vi "Localize CSM VIs.vi"(5 "API Dir":path[](array[path]), 6 "options":cluster{"Force?(F)":bool, "Show FP":bool}={"Force?(F)"=FALSE, "Show FP"=TRUE}, 7 "doc dir":path[](array[path]), 8 "error in (no error)":errorcluster, 10 "Language Ring":string(combo)="English(en-us)") -> (0 "error out":errorcluster)   [LabVIEW 2017, in "csmdoc.lvlib"]
uses:
  csmdoc.lvlib
  BEditor-Localization.vi
  _Typedef/DocElement.ctl
  _Shared/CSM Shared.lvlib
  _tool/_batchEditorDialog/batchEditorDialog.lvlib
  Communicable State Machine.lvlib
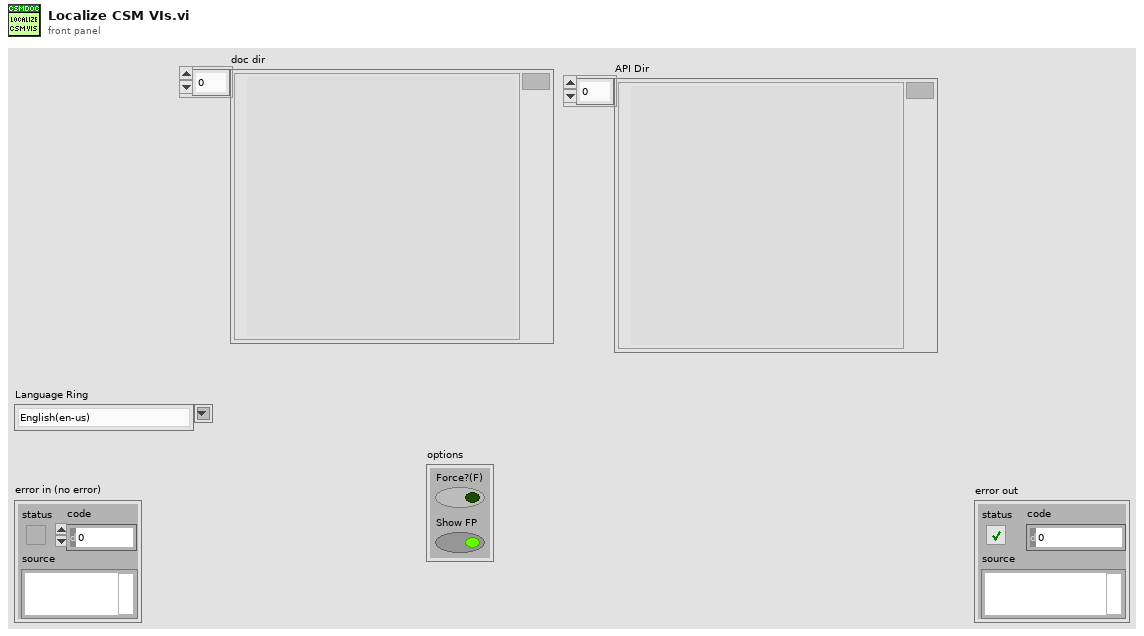
[diagram p1: front panel]
types:
  T1 = typedef "csmdoc.lvlib/DocNote.ctl" = cluster{"ID":string, "Content":string, "Type":string}
  T2 = typedef "csmdoc.lvlib/DocElement.ctl" = cluster{"ID":string, "Content":string[], "SubIDs":string[], "Path":string[]}
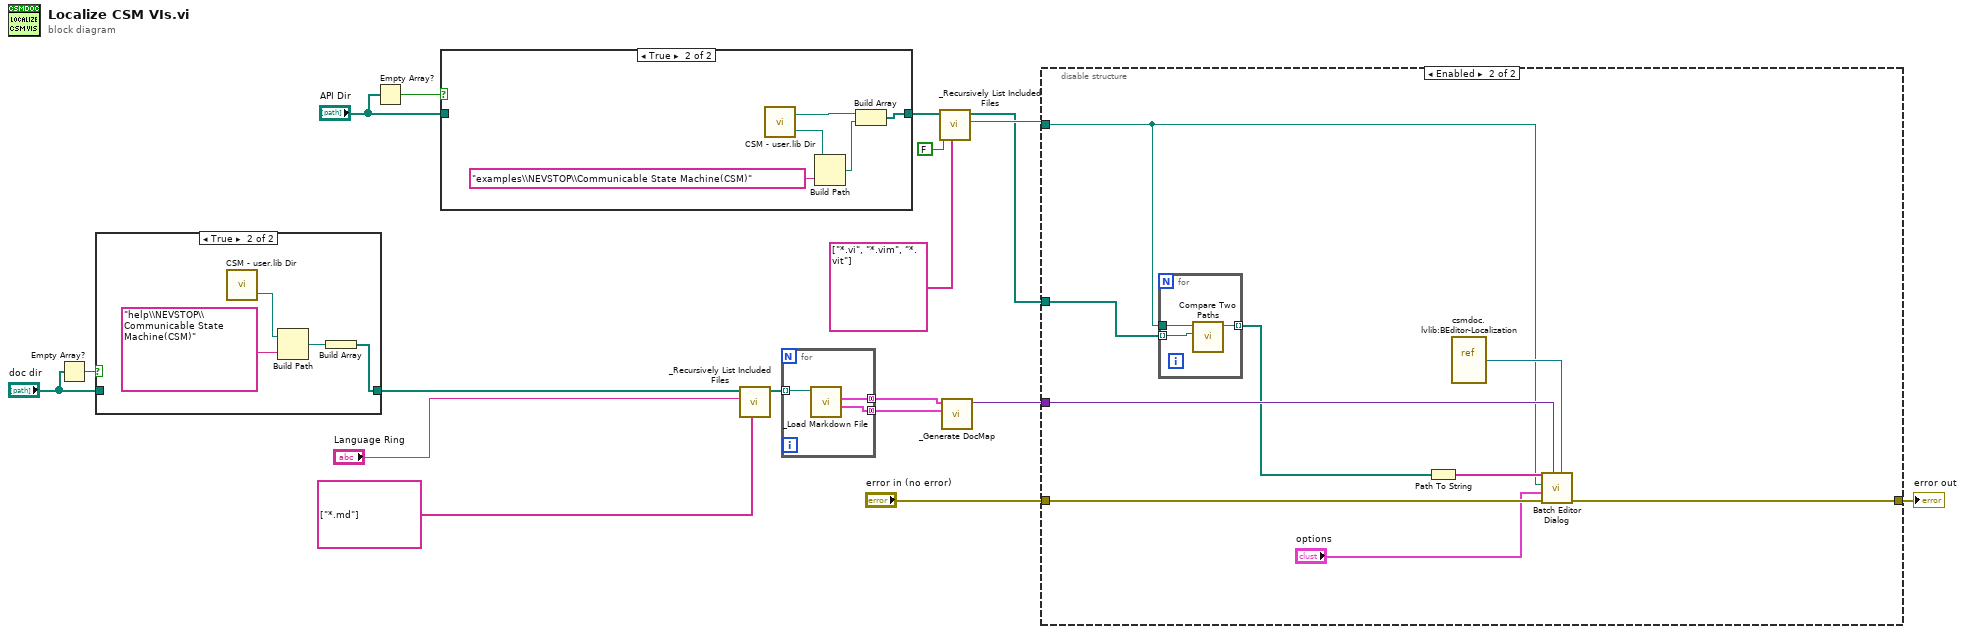
[diagram p0: block diagram]
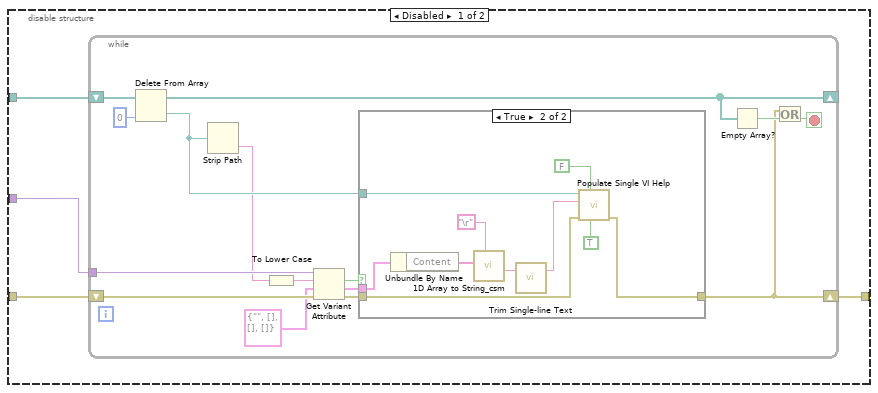
[diagram p2: hidden frame]
diagram:
  n1 = Empty Array?(array="doc dir") -> (empty?=w12:bool)
  n2 = case shown="True" w12 {
    tunnel: [w19 w20] -> w18
    tunnel: "doc dir" -> [w19 _]
    frame False {
    }
    frame True {
      n3 = call "CSM - user.lib Dir.vi"() -> ("<LabVIEW>"=w21:path)  [unwired: 2 in, 1 out]
      n4 = Build Path(base path=w21, name or relative path="help\\NEVSTOP\\Communicable State Machine(CSM)") -> (appended path=w22:path)
      n5 = Build Array(w22) -> (w20:path[])
    }
  }
  n6 = Empty Array?(array="API Dir") -> (empty?=w10:bool)
  n7 = case shown="True" w10 {
    tunnel: "API Dir" -> [w24 _]
    tunnel: [w24 w29] -> w3
    frame False {
    }
    frame True {
      n8 = call "CSM - user.lib Dir.vi"() -> ("<LabVIEW>"=w27:path, "csm_user.lib_dir"=w28:path)  [unwired: 2 in]
      n9 = Build Path(base path=w27, name or relative path="examples\\NEVSTOP\\Communicable State Machine(CSM)") -> (appended path=w25:path)
      n10 = Build Array(w28, w25) -> (w29:path[])
    }
  }
  n11 = call "_Recursively List Included Files.vi"("pattern"=string[] ["*.md"], "Language Ring"="Language Ring", "dir"=w18) -> ("Array"=w15:path[])  [unwired: 7 in, 1 out]
  n12 = for {
    tunnel: w15 -> [w32] mode=indexing
    tunnel: [w31] -> w17 mode=concatenating
    tunnel: [w30] -> w16 mode=concatenating
    n13 = call "_Load Markdown File.vi"("Path"=w32) -> ("Array 2"=w30:T1[], "Array"=w31:T2[])  [unwired: 8 in, 1 out]
  }
  n14 = call "_Recursively List Included Files.vi"("pattern"=string[] ["*.vi", "*.vim", "*.vit"], "apply _ filter?(T)"=FALSE, "dir"=w3) -> ("Common Path"=w6:path, "Array"=w4:path[])  [unwired: 7 in]
  n15 = call "_Generate DocMap.vi"("Array 2"=w16, "Array"=w17) -> ("Variant"=w13:variant)  [unwired: 9 in]
  n16 = disable-structure shown="Enabled" {
    disable-tunnel: [w36 w70] -> w14
    disable-tunnel: "error in (no error)" -> [w35 w71]
    disable-tunnel: w13 -> [w34 w69]
    disable-tunnel: w4 -> [w33 w65]
    disable-tunnel: w6 -> [_ w63]
    frame Disabled {
      n17 = while {
        shift-right: [w48] -> _
        shift-left: w33 -> [w50]
        tunnel: w34 -> [w46]
        shift-right: [w37] -> w36
        shift-left: w35 -> [w43]
        stop <- w38 stop-if-true
        n18 = Delete From Array(array=w50, index=0) -> (deleted portion=w51:path, array with subset deleted=w48:path[])  [unwired: 1 in]
        n19 = Strip Path(path=w51) -> (name=w45:string)  [unwired: 1 out]
        n20 = To Lower Case(string=w45) -> (all lower case string=w40:string)
        n21 = Get Variant Attribute(Variant=w46, name=w40, default value (empty Variant)=T2 {"ID"="", "Content"=[], "SubIDs"=[], "Path"=[]} ("Cluster"), error in=w43) -> (found=w44:bool, value=w41:T2, error out=w42:errorcluster)  [unwired: 1 out]
        n22 = case shown="True" w44 {
          tunnel: w51 -> [_ w62]
          tunnel: w42 -> [w52 w61]
          tunnel: [w52 w60] -> w37
          tunnel: w41 -> [_ w56]
          frame False {
          }
          frame True {
            n23 = Unbundle By Name(w56) -> ("Content"=w59:string[])
            n24 = call "1D Array to String_csm.vi"("delimiter (Tab)"="\r", "Array of Strings"=w59) -> ("delimited string"=w57:string)  [unwired: 9 in]
            n25 = call "Trim Single-line Text.vi"("single-line text"=w57) -> ("trimed text"=w55:string)  [unwired: 2 in]
            n26 = call "Populate Single VI Help.vi"("Show FP"=TRUE, "Force?(F)"=FALSE, "error in (no error)"=w61, "VI Description"=w55, "Path"=w62) -> ("error out"=w60:errorcluster)  [unwired: 6 in]
          }
        }
        n27 = Empty Array?(array=w48) -> (empty?=w49:bool)
        n28 = Or(x=w37, y=w49) -> (x .or. y?=w38:bool)
      }
    }
    frame Enabled {
      n29 = for {
        tunnel: w63 -> [w74]
        tunnel: w65 -> [w73] mode=indexing
        tunnel: [w72] -> w64 mode=indexing
        n30 = call <vilib>:"Compare Two Paths.vi"("Path 2"=w73, "Path 1"=w74) -> ("Relative Path from 1 to 2"=w72:path)  [unwired: 6 in, 3 out]
      }
      n31 = Path To String(path=w64) -> (string=w68:string[])
      n32 = vi-ref "csmdoc.lvlib:BEditor-Localization.vi"() -> (w67:refnum<vi>)
      n33 = call "Batch Editor Dialog.vi"("VI Refnum"=w67, "Reference"=w69, "Error in"=w71, "Option"="options", "Root"=w63, "Entries"=w68) -> ("Error out"=w70:errorcluster)  [unwired: 5 in]
    }
  }
  "error out" <- w14
